vi "Copy .LLB to NI VeriStand dir.vi"(5 "Files Generated by Build":path[](array[path]), 6 "Top Level/Always Included VIs":path[](array[path]), 7 "Destination Path":path, 8 "error in (no error)":errorcluster, 9 "Target Name":string, 10 "Build Specification Name":string, 11 "Project Path":path) -> (0 "error out":errorcluster)   [LabVIEW 2024]
doc: "This VI is called after each run of a build specification. The VI will copy the generated LLB (Engine or System Explorer) into the VeriStand Custom Device folder (...\\Documents\\National Instruments\\NI VeriStand 2013...)."
uses:
  <vilib>/Utility/sysdir.llb/System Directory Type.ctl
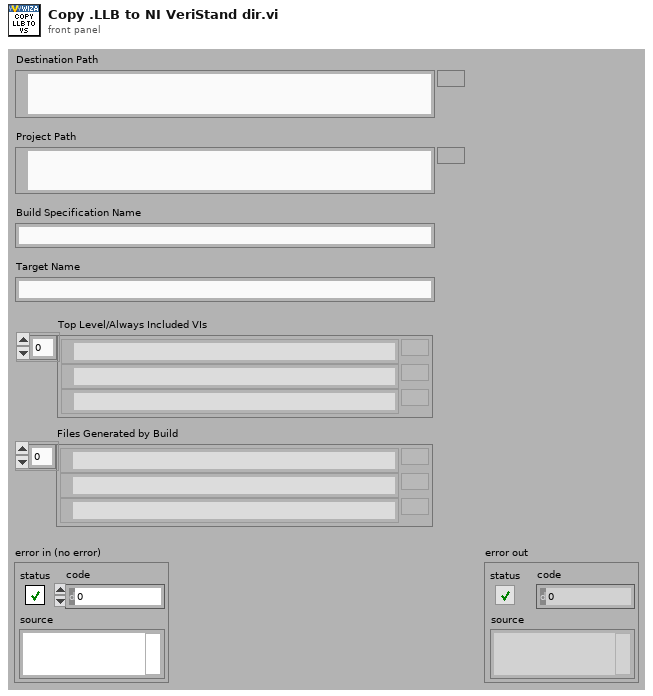
[diagram p1: front panel]
types:
  T1 = typedef "System Directory Type.ctl" = i32
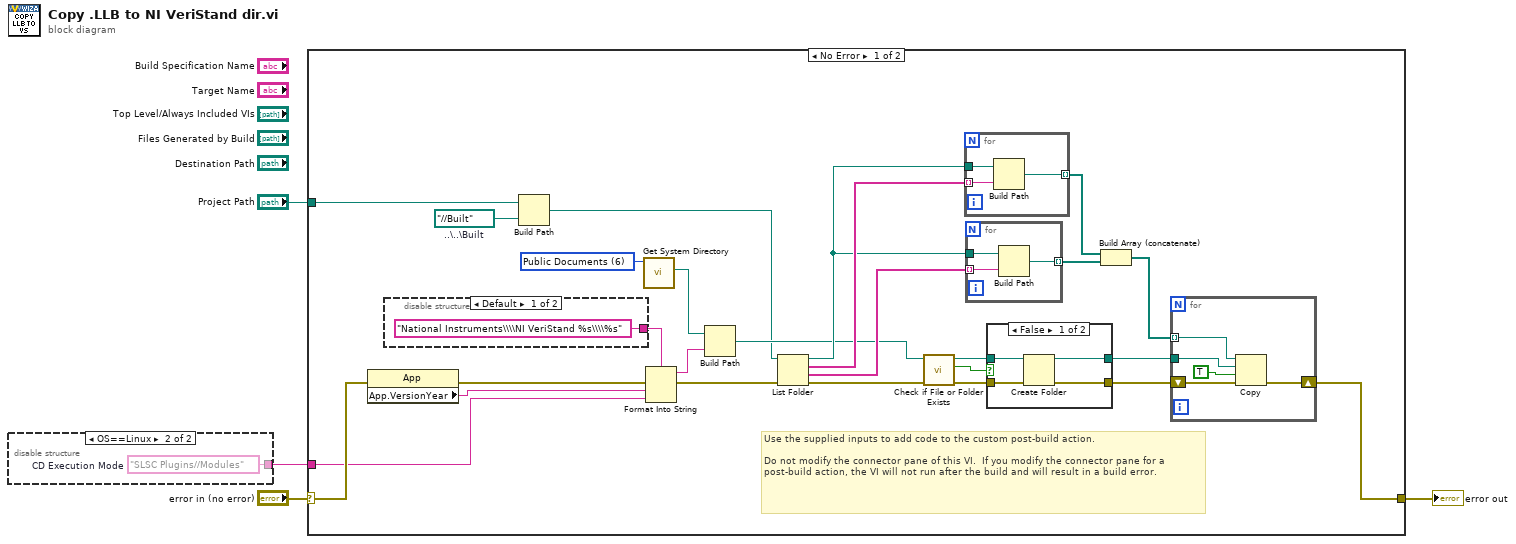
[diagram p0: block diagram]
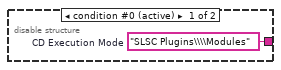
[diagram p2: hidden frame]
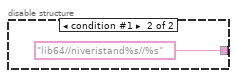
[diagram p3: hidden frame]
diagram:
  n1 = disable-structure shown="OS==Linux" {
    disable-tunnel: [w5 w6] -> w1
    frame condition #0 (active) {
      w5 = "SLSC Plugins\\\\Modules"  # CD Execution Mode
    }
    frame condition #1 {
      w6 = "SLSC Plugins//Modules"  # CD Execution Mode
    }
  }
  n2 = case shown="No Error" "error in (no error)" {
    selector: "error in (no error)" -> [w16 w52]
    tunnel: [w18 w52] -> w2
    tunnel: "Project Path" -> [w14 _]
    tunnel: w1 -> [w8 _]
    frame No Error {
      w7 = path "../../Built"  # ..\..\Built
      w20 = T1 6 items=["User Home"=0, "User Desktop"=1, "User Documents"=2, "User Application Data"=3, "User Preferences"=4, "User Temporary"=5, "Public Documents"=6, "Public Application Data"=7, "Public Preferences"=8, "Public Cache"=13, "System Core Libraries"=9, "System Installed Libraries"=10, "Application Files"=11, "Boot Volume Root"=12] ("system directory type")
      # "Use the supplied inputs to add code to the custom post-build action.\n\nDo not modify the connector pane of this VI.  If you modify the connector pane for a post-build action, the VI will not run after the build and will result in a build error."
      n3 = property class="App"(error in=w16) -> (error out=w19:errorcluster, "App.VersionYear"=w9:string)  [unwired: 1 in, 1 out]
      n4 = disable-structure shown="Default" {
        disable-tunnel: ["National Instruments\\\\NI VeriStand %s\\\\%s" ("name or relative path") "lib64//niveristand%s//%s" ("name or relative path")] -> w10
        frame condition #0 (active) {
        }
        frame condition #1 {
        }
      }
      n5 = Build Path(base path=w14, name or relative path=w7) -> (appended path=w11:path)
      n6 = call <vilib>:"Get System Directory.vi"("system directory type"=w20) -> ("system directory"=w21:path)  [unwired: 10 in]
      n7 = Format Into String(format string=w10, error in=w19, w9, w8) -> (resulting string=w22:string, error out=w15:errorcluster)  [unwired: 1 in]
      n8 = Build Path(base path=w21, name or relative path=w22) -> (appended path=w17:path)
      n9 = List Folder(path=w11, error in=w15) -> (path out=w25:path, filenames=w32:string[], folder names=w26:string[], error out=w23:errorcluster)  [unwired: 2 in]
      n10 = call <vilib>:"Check if File or Folder Exists.vi"("error in (no error)"=w23, "path"=w17) -> ("error out"=w27:errorcluster, "file or folder exists?"=w29:bool, "dup path"=w28:path)  [unwired: 7 in]
      n11 = for {
        tunnel: w32 -> [w50] mode=indexing
        tunnel: w25 -> [w51]
        tunnel: [w49] -> w31 mode=indexing
        n12 = Build Path(base path=w51, name or relative path=w50) -> (appended path=w49:path)
      }
      n13 = for {
        tunnel: w26 -> [w47] mode=indexing
        tunnel: w25 -> [w48]
        tunnel: [w46] -> w24 mode=indexing
        n14 = Build Path(base path=w48, name or relative path=w47) -> (appended path=w46:path)
      }
      n15 = case shown="False" w29 {
        tunnel: w28 -> [w38 w40]
        tunnel: w27 -> [w37 w39]
        tunnel: [w36 w40] -> w13
        tunnel: [w35 w39] -> w12
        frame False {
          n16 = Create Folder(path (use dialog)=w38, error in=w37) -> (created path=w36:path, error out=w35:errorcluster)  [unwired: 1 in, 1 out]
        }
        frame True {
        }
      }
      n17 = Build Array (concatenate)(w31, w24) -> (w30:path[])
      n18 = for {
        tunnel: w30 -> [w42] mode=indexing
        shift-right: [w43] -> w18
        shift-left: w12 -> [w44]
        tunnel: w13 -> [w41]
        n19 = Copy(8:w44, 9:TRUE ("overwrite (F)"), 10:w41, 11:w42) -> (0:w43:errorcluster)  [unwired: 1 in, 2 out]
      }
    }
    frame Error {
    }
  }
  "error out" <- w2
